vi "ZM-CP-close.vi"(8 "error in (no error)":errorcluster, 11 "ZM-CP-UDP-receiver in":refnum<class "ZM-CP-UDP-receiver.lvclass">) -> (0 "error out":errorcluster, 3 "ZM-CP-UDP-receiver out":refnum<class "ZM-CP-UDP-receiver.lvclass">)   [LabVIEW 2020, in "ZM-CP-UDP-udp_transport.lvlib" / "ZM-CP-UDP-receiver.lvclass"]
doc: "Closes the communication protocol (dynamic dispatch): writes opened = FALSE through the private accessor Write opened. This is the real default of the parent; a child that holds resources runs its own hook and then calls the parent."
uses:
  ZM-CP-UDP-receiver.lvclass
  ZM-CP-communication_protocol/ZM-CP-communication_protocol/ZM-CP-communication_protocol.lvclass
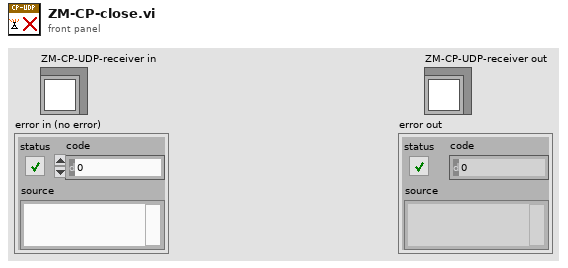
[diagram p1: front panel]
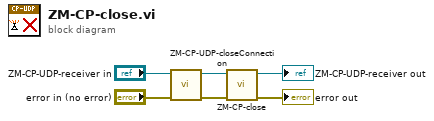
[diagram p0: block diagram]
diagram:
  n1 = call "ZM-CP-UDP-closeConnection.vi"("error in (no error)"="error in (no error)", "ZM-CP-communication_protocol in"="ZM-CP-UDP-receiver in") -> ("error out"=w1:errorcluster, "ZM-CP-communication_protocol out"=w3:refnum<class "ZM-CP-UDP-receiver.lvclass">)  [unwired: 8 in]
  n2 = call-parent "ZM-CP-close.vi"("error in (no error)"=w1, "ZM-CP-communication_protocol in"=w3) -> ("error out"=→"error out":errorcluster, "ZM-CP-communication_protocol out"=→"ZM-CP-UDP-receiver out":refnum<class "ZM-CP-UDP-receiver.lvclass">)  [unwired: 8 in]
